vi "toString.vi"(10 "Variant":variant, 11 "StringFormatter in":refnum<class "StringFormatter.lvclass">) -> (2 "Value":string)   [LabVIEW 2013, in "OpenStringFormatter.lvlib" / "StringFormatter.lvclass"]
uses:
  StringFormatter.lvclass
  StringFormatter.lvclass/StringFormatter.ctl
  <vilib>/Utility/GetType.llb/TD_MDTFlavor.ctl
  TypeDescriptor/OpenDescriptor.lvlib
  Conversions/OpenConvert.lvlib
  Variant/OpenVariant.lvlib
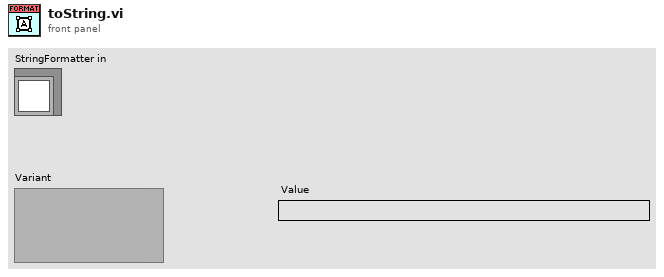
[diagram p1: front panel]
types:
  T1 = typedef "OpenStringFormatter.lvlib/StringFormatter.lvclass/Localization Decimal Separator -- enum.ctl" = enum16{"System", "Comma", "Dot"}
  T2 = typedef "VariantType.lvlib/UnitInfo.ctl" = cluster{"UnitType":T3, "Exponent":i16}
  T3 = typedef "VariantType.lvlib/UnitType.ctl" = enum16{"Radians", "Steradians", "Seconds", "Meters", "Kilograms", "Amperes", "Kelvins", "Moles", "Candelas", "InvalidUnit"}
  T4 = typedef "TD_Refnum Kind.ctl" = enum16{"Generic", "DataLog", "ByteStream", "Device", "Occur", "TCPNetConn", "OldVisa", "Auto", "LVObj", "Menu", "OldIVI", "Imaq", "Hardware", "DataSocket", "Visa", "IVI", "UDPNetConn", "Notifier", "Queue", "IrdaNetConn", "GenClass", "GenClassTag", "DAQMX", "EventReg", "DotNet", "UserEvent", "GenClassDeepCopy", "Callback", "GenClassFlatten", "GenClassTagFlatten", "LV Class Instance", "BtNetConn"}
  T5 = typedef "TD_MDTFlavor.ctl" = enum16{"kUnknown", "OldDblWaveform", "I16Waveform", "DBLWaveform", "Unused(4)", "SGLWaveform", "Timestamp", "DigitalTable", "DigitalWaveform", "Dynamic Express", "ExtWaveform", "U8Waveform", "U16Waveform", "U32Waveform", "I8Waveform", "I32Waveform", "CSGWaveform", "CDBWaveform", "CXTWaveform", "I64Waveform", "U64Waveform"}
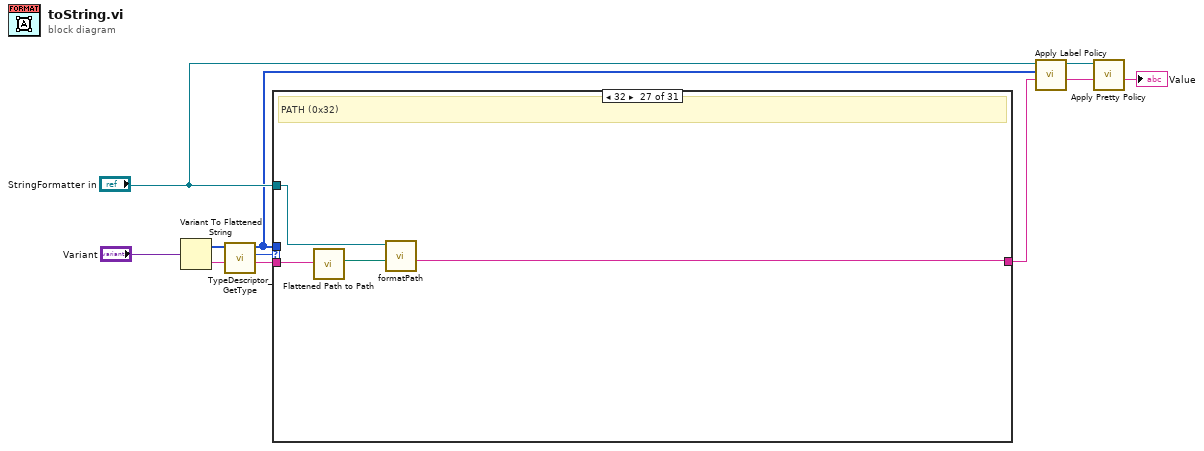
[diagram p0: block diagram]
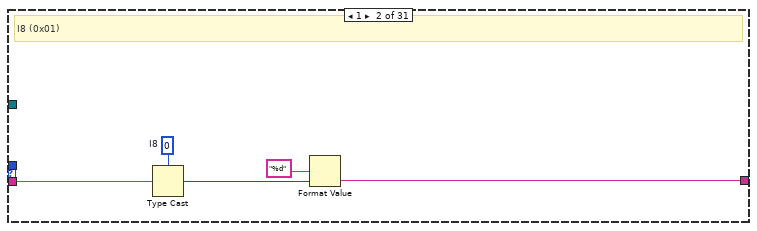
[diagram p3: hidden frame]
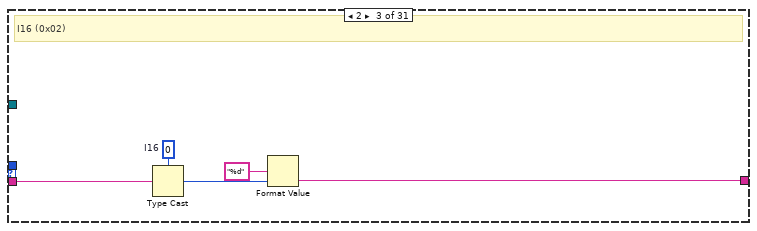
[diagram p4: hidden frame]
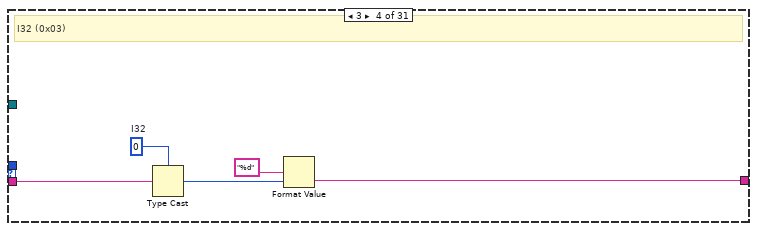
[diagram p5: hidden frame]
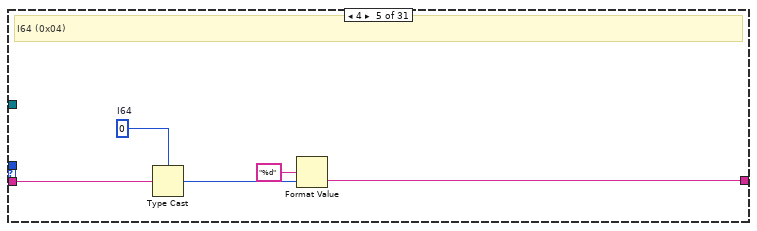
[diagram p6: hidden frame]
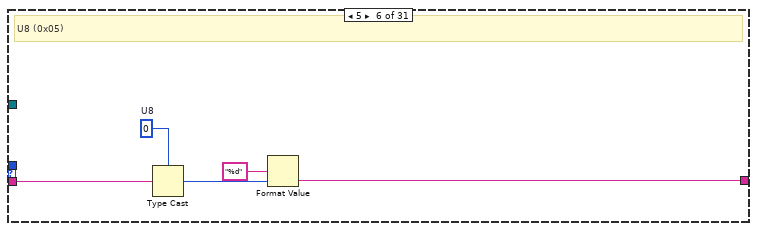
[diagram p7: hidden frame]
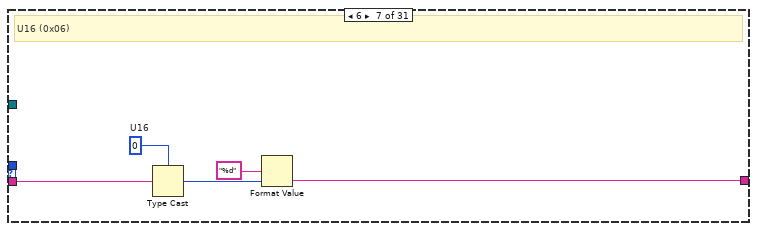
[diagram p8: hidden frame]
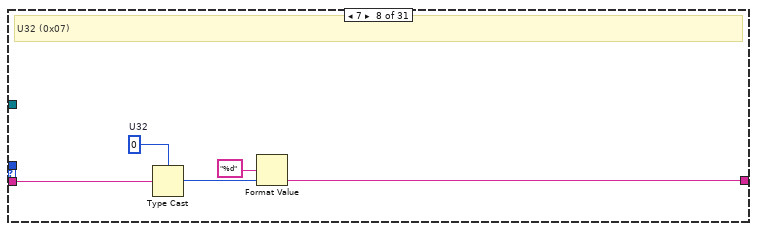
[diagram p9: hidden frame]
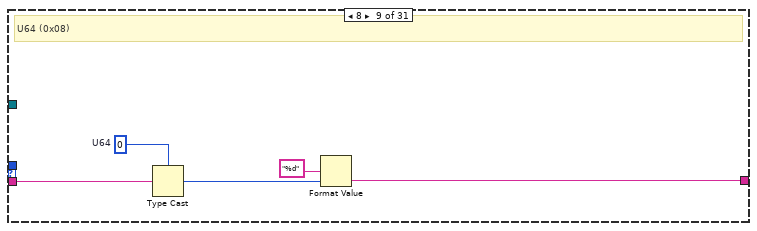
[diagram p10: hidden frame]
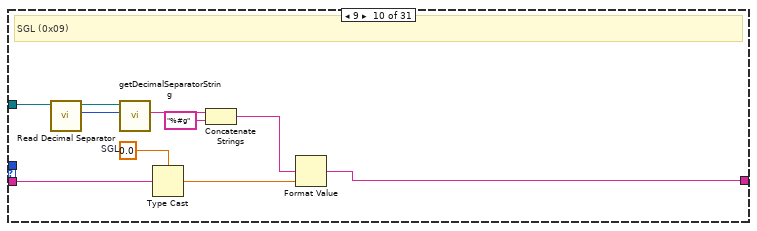
[diagram p11: hidden frame]
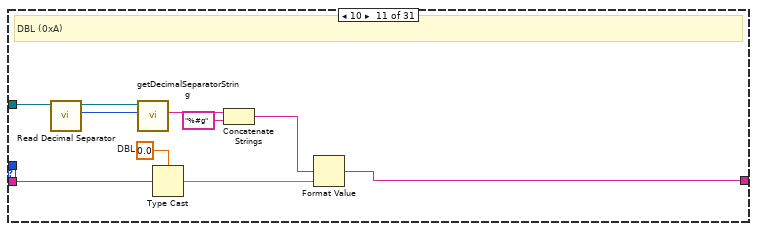
[diagram p12: hidden frame]
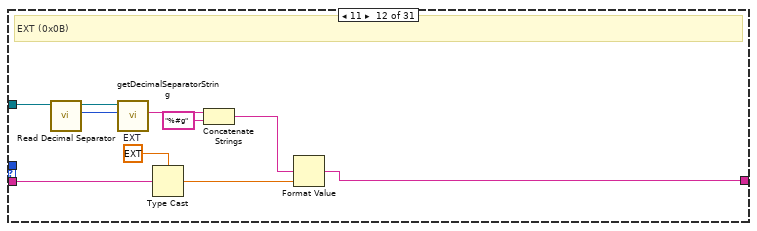
[diagram p13: hidden frame]
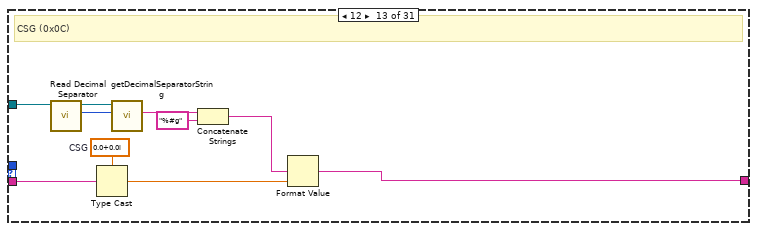
[diagram p14: hidden frame]
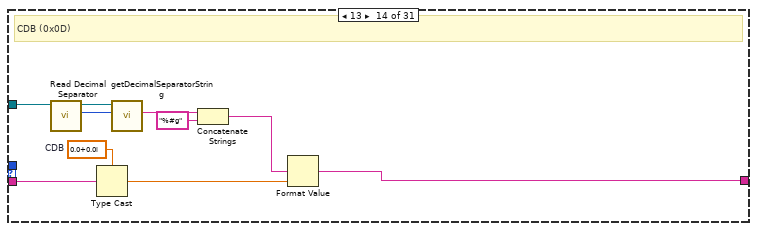
[diagram p15: hidden frame]
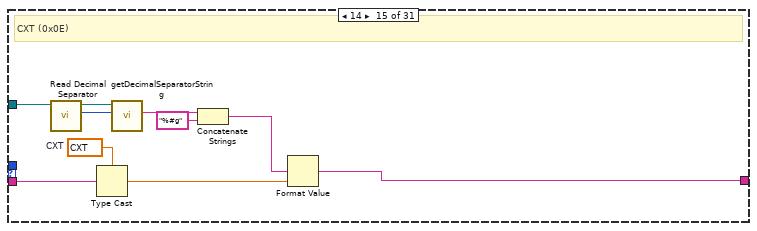
[diagram p16: hidden frame]
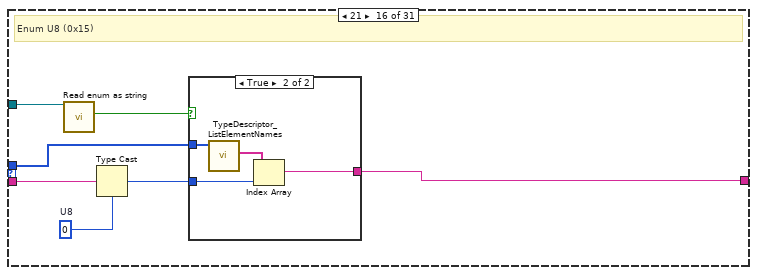
[diagram p17: hidden frame]
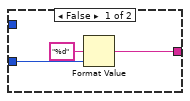
[diagram p18: hidden frame]
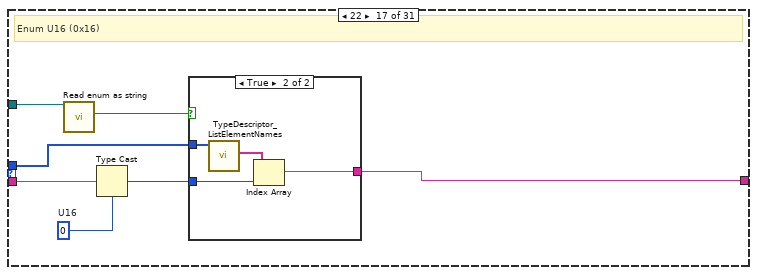
[diagram p19: hidden frame]
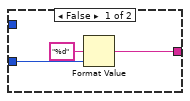
[diagram p20: hidden frame]
diagram:
  n1 = Variant To Flattened String(Variant="Variant") -> (data string=w8:string, 1:w10:i16[])
  n2 = call "TypeDescriptor_GetType.vi"("type descriptor"=w10) -> ("Type"=w9:u8, "type descriptor dup"=w5:i16[])  [unwired: 9 in]
  n3 = case shown="32" w9 {
    tunnel: [_ w11 w16 w21 w26 w31 w36 w41 w46 w52 w62 w72 w86 w97 w107 w115 w129 w143 w157 w173 w188 w203 w218 w233 w243 w250 w253 w257 w279 w303 w324] -> w4
    tunnel: w8 -> [_ w15 w19 w24 w29 w34 w39 w44 w49 w58 w69 w79 w89 w99 w109 w117 w131 w145 w167 w182 w197 w212 w227 w242 w248 w252 w256 w273 w291 w304 w325]
    tunnel: "StringFormatter in" -> [_ _ _ _ _ _ _ _ _ w59 w70 w80 w90 w100 w110 w113 w127 w140 w162 w178 w193 w208 w223 w238 _ w249 w254 w259 w281 w302 w323]
    tunnel: w5 -> [_ _ _ _ _ _ _ _ _ _ _ _ _ _ _ w114 w128 w141 w160 w176 w191 w206 w221 w236 _ _ _ w258 w280 w306 w322]
    frame 0, Default {
      # "Default"
    }
    frame 1 {
      w14 = i8 0  # I8
      # "I8 (0x01)"
      n4 = Type Cast(type=w14, x=w15) -> (*(type *) &x=w12:i8)
      n5 = Format Value(format string="%d", value (0)=w12) -> (output string=w11:string)  [unwired: 1 in]
    }
    frame 2 {
      w20 = i16 0  # I16
      # "I16 (0x02)"
      n6 = Type Cast(type=w20, x=w19) -> (*(type *) &x=w17:i16)
      n7 = Format Value(format string="%d", value (0)=w17) -> (output string=w16:string)  [unwired: 1 in]
    }
    frame 3 {
      w25 = 0  # I32
      # "I32 (0x03)"
      n8 = Type Cast(type=w25, x=w24) -> (*(type *) &x=w22:i32)
      n9 = Format Value(format string="%d", value (0)=w22) -> (output string=w21:string)  [unwired: 1 in]
    }
    frame 4 {
      w30 = i64 0  # I64
      # "I64 (0x04)"
      n10 = Type Cast(type=w30, x=w29) -> (*(type *) &x=w27:i64)
      n11 = Format Value(format string="%d", value (0)=w27) -> (output string=w26:string)  [unwired: 1 in]
    }
    frame 5 {
      w35 = u8 0  # U8
      # "U8 (0x05)"
      n12 = Type Cast(type=w35, x=w34) -> (*(type *) &x=w32:u8)
      n13 = Format Value(format string="%d", value (0)=w32) -> (output string=w31:string)  [unwired: 1 in]
    }
    frame 6 {
      w40 = u16 0  # U16
      # "U16 (0x06)"
      n14 = Type Cast(type=w40, x=w39) -> (*(type *) &x=w37:u16)
      n15 = Format Value(format string="%d", value (0)=w37) -> (output string=w36:string)  [unwired: 1 in]
    }
    frame 7 {
      w45 = u32 0  # U32
      # "U32 (0x07)"
      n16 = Type Cast(type=w45, x=w44) -> (*(type *) &x=w42:u32)
      n17 = Format Value(format string="%d", value (0)=w42) -> (output string=w41:string)  [unwired: 1 in]
    }
    frame 8 {
      w50 = u64 0  # U64
      # "U64 (0x08)"
      n18 = Type Cast(type=w50, x=w49) -> (*(type *) &x=w47:u64)
      n19 = Format Value(format string="%d", value (0)=w47) -> (output string=w46:string)  [unwired: 1 in]
    }
    frame 9 {
      w60 = sgl 0.0  # SGL
      # "SGL (0x09)"
      n20 = call "Read Decimal Separator.vi"("StringFormatter in"=w59) -> ("Decimal Separator"=w54:T1, "StringFormatter out"=w51:refnum<class "StringFormatter.lvclass">)  [unwired: 9 in]
      n21 = call-dynamic "getDecimalSeparatorString.vi"("Decimal Separator"=w54, "StringFormatter"=w51) -> ("Formatter String"=w57:string)  [unwired: 9 in]
      n22 = Type Cast(type=w60, x=w58) -> (*(type *) &x=w53:sgl)
      n23 = Concatenate Strings(w57, "%#g" ("string")) -> (w56:string)
      n24 = Format Value(format string=w56, value (0)=w53) -> (output string=w52:string)  [unwired: 1 in]
    }
    frame 10 {
      w68 = 0.0  # DBL
      # "DBL (0xA)"
      n25 = call "Read Decimal Separator.vi"("StringFormatter in"=w70) -> ("Decimal Separator"=w64:T1, "StringFormatter out"=w61:refnum<class "StringFormatter.lvclass">)  [unwired: 9 in]
      n26 = call-dynamic "getDecimalSeparatorString.vi"("Decimal Separator"=w64, "StringFormatter"=w61) -> ("Formatter String"=w67:string)  [unwired: 9 in]
      n27 = Type Cast(type=w68, x=w69) -> (*(type *) &x=w63:dbl)
      n28 = Concatenate Strings(w67, "%#g" ("string")) -> (w66:string)
      n29 = Format Value(format string=w66, value (0)=w63) -> (output string=w62:string)  [unwired: 1 in]
    }
    frame 11 {
      w78 = ext 0.0  # EXT
      # "EXT (0x0B)"
      n30 = call "Read Decimal Separator.vi"("StringFormatter in"=w80) -> ("Decimal Separator"=w74:T1, "StringFormatter out"=w71:refnum<class "StringFormatter.lvclass">)  [unwired: 9 in]
      n31 = call-dynamic "getDecimalSeparatorString.vi"("Decimal Separator"=w74, "StringFormatter"=w71) -> ("Formatter String"=w77:string)  [unwired: 9 in]
      n32 = Type Cast(type=w78, x=w79) -> (*(type *) &x=w73:ext)
      n33 = Concatenate Strings(w77, "%#g" ("string")) -> (w76:string)
      n34 = Format Value(format string=w76, value (0)=w73) -> (output string=w72:string)  [unwired: 1 in]
    }
    frame 12 {
      w88 = csg 0.0+0.0i  # CSG
      # "CSG (0x0C)"
      n35 = call "Read Decimal Separator.vi"("StringFormatter in"=w90) -> ("Decimal Separator"=w85:T1, "StringFormatter out"=w81:refnum<class "StringFormatter.lvclass">)  [unwired: 9 in]
      n36 = Type Cast(type=w88, x=w89) -> (*(type *) &x=w87:csg)
      n37 = call-dynamic "getDecimalSeparatorString.vi"("Decimal Separator"=w85, "StringFormatter"=w81) -> ("Formatter String"=w84:string)  [unwired: 9 in]
      n38 = Concatenate Strings(w84, "%#g" ("string")) -> (w83:string)
      n39 = Format Value(format string=w83, value (0)=w87) -> (output string=w86:string)  [unwired: 1 in]
    }
    frame 13 {
      w92 = cdb 0.0+0.0i  # CDB
      # "CDB (0x0D)"
      n40 = call "Read Decimal Separator.vi"("StringFormatter in"=w100) -> ("Decimal Separator"=w96:T1, "StringFormatter out"=w91:refnum<class "StringFormatter.lvclass">)  [unwired: 9 in]
      n41 = Type Cast(type=w92, x=w99) -> (*(type *) &x=w98:cdb)
      n42 = call-dynamic "getDecimalSeparatorString.vi"("Decimal Separator"=w96, "StringFormatter"=w91) -> ("Formatter String"=w95:string)  [unwired: 9 in]
      n43 = Concatenate Strings(w95, "%#g" ("string")) -> (w94:string)
      n44 = Format Value(format string=w94, value (0)=w98) -> (output string=w97:string)  [unwired: 1 in]
    }
    frame 14 {
      w102 = cxt 0.0+0.0i  # CXT
      # "CXT (0x0E)"
      n45 = call "Read Decimal Separator.vi"("StringFormatter in"=w110) -> ("Decimal Separator"=w106:T1, "StringFormatter out"=w101:refnum<class "StringFormatter.lvclass">)  [unwired: 9 in]
      n46 = Type Cast(type=w102, x=w109) -> (*(type *) &x=w108:cxt)
      n47 = call-dynamic "getDecimalSeparatorString.vi"("Decimal Separator"=w106, "StringFormatter"=w101) -> ("Formatter String"=w105:string)  [unwired: 9 in]
      n48 = Concatenate Strings(w105, "%#g" ("string")) -> (w104:string)
      n49 = Format Value(format string=w104, value (0)=w108) -> (output string=w107:string)  [unwired: 1 in]
    }
    frame 21 {
      w111 = u8 0  # U8
      # "Enum U8 (0x15)"
      n50 = call "Read enum as string.vi"("StringFormatter in"=w113) -> ("enum as string"=w112:bool)  [unwired: 9 in, 1 out]
      n51 = Type Cast(type=w111, x=w117) -> (*(type *) &x=w116:u8)
      n52 = case shown="True" w112 {
        tunnel: w116 -> [w120 w122]
        tunnel: [w119 w121] -> w115
        tunnel: w114 -> [_ w124]
        frame False {
          n53 = Format Value(format string="%d", value (0)=w120) -> (output string=w119:string)  [unwired: 1 in]
        }
        frame True {
          n54 = call "TypeDescriptor_ListElementNames.vi"("type descriptor"=w124) -> ("element names"=w123:string[])  [unwired: 7 in, 3 out]
          n55 = Index Array(array=w123, index=w122) -> (element=w121:string)
        }
      }
    }
    frame 22 {
      w125 = u16 0  # U16
      # "Enum U16 (0x16)"
      n56 = call "Read enum as string.vi"("StringFormatter in"=w127) -> ("enum as string"=w126:bool)  [unwired: 9 in, 1 out]
      n57 = Type Cast(type=w125, x=w131) -> (*(type *) &x=w130:u16)
      n58 = case shown="True" w126 {
        tunnel: w130 -> [w134 w136]
        tunnel: [w133 w135] -> w129
        tunnel: w128 -> [_ w138]
        frame False {
          n59 = Format Value(format string="%d", value (0)=w134) -> (output string=w133:string)  [unwired: 1 in]
        }
        frame True {
          n60 = call "TypeDescriptor_ListElementNames.vi"("type descriptor"=w138) -> ("element names"=w137:string[])  [unwired: 7 in, 3 out]
          n61 = Index Array(array=w137, index=w136) -> (element=w135:string)
        }
      }
    }
    frame 23 {
      w142 = u32 0  # U32
      # "Enum U32 (0x17)"
      n62 = call "Read enum as string.vi"("StringFormatter in"=w140) -> ("enum as string"=w139:bool)  [unwired: 9 in, 1 out]
      n63 = Type Cast(type=w142, x=w145) -> (*(type *) &x=w144:u32)
      n64 = case shown="True" w139 {
        tunnel: w144 -> [w148 w150]
        tunnel: [w147 w149] -> w143
        tunnel: w141 -> [_ w152]
        frame False {
          n65 = Format Value(format string="%d", value (0)=w148) -> (output string=w147:string)  [unwired: 1 in]
        }
        frame True {
          n66 = call "TypeDescriptor_ListElementNames.vi"("type descriptor"=w152) -> ("element names"=w151:string[])  [unwired: 7 in, 3 out]
          n67 = Index Array(array=w151, index=w150) -> (element=w149:string)
        }
      }
    }
    frame 25 {
      w165 = sgl 0.0  # SGL
      # "SGL PhysUnit (0x19)"
      n68 = call "Read Decimal Separator.vi"("StringFormatter in"=w162) -> ("Decimal Separator"=w161:T1, "StringFormatter out"=w153:refnum<class "StringFormatter.lvclass">)  [unwired: 9 in]
      n69 = call "TypeDescriptor_GetUnits.vi"("type descriptor"=w160) -> ("Units"=w155:T2[])  [unwired: 8 in, 2 out]
      n70 = Type Cast(type=w165, x=w167) -> (*(type *) &x=w166:sgl)
      n71 = call-dynamic "formatUnits.vi"("Units"=w155, "StringFormatter"=w153) -> ("Units String"=w154:string)  [unwired: 9 in]
      n72 = call-dynamic "getDecimalSeparatorString.vi"("Decimal Separator"=w161, "StringFormatter"=w153) -> ("Formatter String"=w164:string)  [unwired: 9 in]
      n73 = Concatenate Strings(w164, "%#g" ("string")) -> (w159:string)
      n74 = Format Value(format string=w159, value (0)=w166) -> (output string=w158:string)  [unwired: 1 in]
      n75 = call <vilib>:"Space Constant.vi"() -> ("String"=w156:string)
      n76 = Concatenate Strings(w158, w156, w154) -> (w157:string)
    }
    frame 26 {
      w168 = 0.0  # DBL
      # "DBL PhysUnit (0x1A)"
      n77 = call "Read Decimal Separator.vi"("StringFormatter in"=w178) -> ("Decimal Separator"=w177:T1, "StringFormatter out"=w169:refnum<class "StringFormatter.lvclass">)  [unwired: 9 in]
      n78 = call "TypeDescriptor_GetUnits.vi"("type descriptor"=w176) -> ("Units"=w171:T2[])  [unwired: 8 in, 2 out]
      n79 = Type Cast(type=w168, x=w182) -> (*(type *) &x=w181:dbl)
      n80 = call-dynamic "formatUnits.vi"("Units"=w171, "StringFormatter"=w169) -> ("Units String"=w170:string)  [unwired: 9 in]
      n81 = call-dynamic "getDecimalSeparatorString.vi"("Decimal Separator"=w177, "StringFormatter"=w169) -> ("Formatter String"=w180:string)  [unwired: 9 in]
      n82 = Concatenate Strings(w180, "%#g" ("string")) -> (w175:string)
      n83 = Format Value(format string=w175, value (0)=w181) -> (output string=w174:string)  [unwired: 1 in]
      n84 = call <vilib>:"Space Constant.vi"() -> ("String"=w172:string)
      n85 = Concatenate Strings(w174, w172, w170) -> (w173:string)
    }
    frame 27 {
      w183 = ext 0.0  # EXT
      # "EXT PhysUnit (0x1B)"
      n86 = call "Read Decimal Separator.vi"("StringFormatter in"=w193) -> ("Decimal Separator"=w192:T1, "StringFormatter out"=w184:refnum<class "StringFormatter.lvclass">)  [unwired: 9 in]
      n87 = call "TypeDescriptor_GetUnits.vi"("type descriptor"=w191) -> ("Units"=w186:T2[])  [unwired: 8 in, 2 out]
      n88 = Type Cast(type=w183, x=w197) -> (*(type *) &x=w196:ext)
      n89 = call-dynamic "formatUnits.vi"("Units"=w186, "StringFormatter"=w184) -> ("Units String"=w185:string)  [unwired: 9 in]
      n90 = call-dynamic "getDecimalSeparatorString.vi"("Decimal Separator"=w192, "StringFormatter"=w184) -> ("Formatter String"=w195:string)  [unwired: 9 in]
      n91 = Concatenate Strings(w195, "%#g" ("string")) -> (w190:string)
      n92 = Format Value(format string=w190, value (0)=w196) -> (output string=w189:string)  [unwired: 1 in]
      n93 = call <vilib>:"Space Constant.vi"() -> ("String"=w187:string)
      n94 = Concatenate Strings(w189, w187, w185) -> (w188:string)
    }
    frame 28 {
      w198 = csg 0.0+0.0i  # CSG
      # "CSG PhysUnit (0x1C)"
      n95 = call "Read Decimal Separator.vi"("StringFormatter in"=w208) -> ("Decimal Separator"=w207:T1, "StringFormatter out"=w199:refnum<class "StringFormatter.lvclass">)  [unwired: 9 in]
      n96 = call "TypeDescriptor_GetUnits.vi"("type descriptor"=w206) -> ("Units"=w201:T2[])  [unwired: 8 in, 2 out]
      n97 = Type Cast(type=w198, x=w212) -> (*(type *) &x=w211:csg)
      n98 = call-dynamic "formatUnits.vi"("Units"=w201, "StringFormatter"=w199) -> ("Units String"=w200:string)  [unwired: 9 in]
      n99 = call-dynamic "getDecimalSeparatorString.vi"("Decimal Separator"=w207, "StringFormatter"=w199) -> ("Formatter String"=w210:string)  [unwired: 9 in]
      n100 = Concatenate Strings(w210, "%#g" ("string")) -> (w205:string)
      n101 = Format Value(format string=w205, value (0)=w211) -> (output string=w204:string)  [unwired: 1 in]
      n102 = call <vilib>:"Space Constant.vi"() -> ("String"=w202:string)
      n103 = Concatenate Strings(w204, w202, w200) -> (w203:string)
    }
    frame 29 {
      w213 = cdb 0.0+0.0i  # CDB
      # "CDB PhysUnit (0x1D)"
      n104 = call "Read Decimal Separator.vi"("StringFormatter in"=w223) -> ("Decimal Separator"=w222:T1, "StringFormatter out"=w214:refnum<class "StringFormatter.lvclass">)  [unwired: 9 in]
      n105 = call "TypeDescriptor_GetUnits.vi"("type descriptor"=w221) -> ("Units"=w216:T2[])  [unwired: 8 in, 2 out]
      n106 = Type Cast(type=w213, x=w227) -> (*(type *) &x=w226:cdb)
      n107 = call-dynamic "formatUnits.vi"("Units"=w216, "StringFormatter"=w214) -> ("Units String"=w215:string)  [unwired: 9 in]
      n108 = call-dynamic "getDecimalSeparatorString.vi"("Decimal Separator"=w222, "StringFormatter"=w214) -> ("Formatter String"=w225:string)  [unwired: 9 in]
      n109 = Concatenate Strings(w225, "%#g" ("string")) -> (w220:string)
      n110 = Format Value(format string=w220, value (0)=w226) -> (output string=w219:string)  [unwired: 1 in]
      n111 = call <vilib>:"Space Constant.vi"() -> ("String"=w217:string)
      n112 = Concatenate Strings(w219, w217, w215) -> (w218:string)
    }
    frame 30 {
      w228 = cxt 0.0+0.0i  # CXT
      # "CXT PhysUnit (0x1E)"
      n113 = call "Read Decimal Separator.vi"("StringFormatter in"=w238) -> ("Decimal Separator"=w237:T1, "StringFormatter out"=w229:refnum<class "StringFormatter.lvclass">)  [unwired: 9 in]
      n114 = call "TypeDescriptor_GetUnits.vi"("type descriptor"=w236) -> ("Units"=w231:T2[])  [unwired: 8 in, 2 out]
      n115 = Type Cast(type=w228, x=w242) -> (*(type *) &x=w241:cxt)
      n116 = call-dynamic "formatUnits.vi"("Units"=w231, "StringFormatter"=w229) -> ("Units String"=w230:string)  [unwired: 9 in]
      n117 = call-dynamic "getDecimalSeparatorString.vi"("Decimal Separator"=w237, "StringFormatter"=w229) -> ("Formatter String"=w240:string)  [unwired: 9 in]
      n118 = Concatenate Strings(w240, "%#g" ("string")) -> (w235:string)
      n119 = Format Value(format string=w235, value (0)=w241) -> (output string=w234:string)  [unwired: 1 in]
      n120 = call <vilib>:"Space Constant.vi"() -> ("String"=w232:string)
      n121 = Concatenate Strings(w234, w232, w230) -> (w233:string)
    }
    frame 33 {
      # "Boolean (0x21)"
      n122 = Type Cast(type=FALSE, x=w248) -> (*(type *) &x=w246:bool)
      n123 = Select(t="true", s=w246, f="false") -> (s? t:f=w243:string)
    }
    frame 48 {
      # "STRING (0x30)"
      n124 = call "Flattened String to String.vi"("Flattened String"=w252) -> ("String"=w251:string)  [unwired: 9 in, 1 out]
      n125 = call-dynamic "formatString.vi"("Value"=w251, "StringFormatter"=w249) -> ("Formatted Value"=w250:string)  [unwired: 9 in]
    }
    frame 50 {
      # "PATH (0x32)"
      n126 = call "Flattened Path to Path.vi"("Flattened Path String"=w256) -> ("path"=w255:path)  [unwired: 10 in]
      n127 = call-dynamic "formatPath.vi"("Value"=w255, "StringFormatter"=w254) -> ("Formatted Value"=w253:string)  [unwired: 9 in]
    }
    frame 64 {
      # "ARRAY (0x40)"
      n128 = call "Write quoted string.vi"("quoted string"=TRUE, "StringFormatter in"=w259) -> ("StringFormatter out"=w261:refnum<class "StringFormatter.lvclass">)  [unwired: 9 in]
      n129 = call "Flattened Array to Flattened Elements.vi"("Flattened Array String"=w273, "Array Type Descriptor"=w258) -> ("Flattened Array Elements"=w271:string[], "Array Element Type Descriptor"=w272:i16[])  [unwired: 8 in]
      n130 = call "Write label.vi"("label"=FALSE, "StringFormatter in"=w261) -> ("StringFormatter out"=w260:refnum<class "StringFormatter.lvclass">)  [unwired: 9 in]
      n131 = for {
        tunnel: w260 -> [w275]
        tunnel: w272 -> [w278]
        tunnel: w271 -> [w277] mode=indexing
        tunnel: [w274] -> w270 mode=indexing
        n132 = Flattened String To Variant(6:w277, 7:w278) -> (3:w276:variant)  [unwired: 1 in, 1 out]
        n133 = call "Variant_FormatToString.vi"("Formatter"=w275, "Variant"=w276) -> ("Value"=w274:string)  [unwired: 9 in]
      }
      n134 = Array To Spreadsheet String(delimiter (Tab)=",", array=w270, 3:"" ("format string")) -> (spreadsheet string=w267:string)
      n135 = call <vilib>:"Trim Whitespace.vi"("string"=w267) -> ("trimmed string"=w266:string)  [unwired: 1 in]
      n136 = Concatenate Strings("[", w266, "]") -> (w257:string)
    }
    frame 80 {
      # "CLUSTER (0x50)"
      n137 = call "Write quoted string.vi"("quoted string"=TRUE, "StringFormatter in"=w281) -> ("StringFormatter out"=w287:refnum<class "StringFormatter.lvclass">)  [unwired: 9 in]
      n138 = call "Flattened Cluster to Flattened Elements.vi"("Flattened Cluster"=w291, "Cluster Type Descriptor"=w280) -> ("Flattened Cluster Elements"=w289:string[], "Elements Type Descriptor"=w290:cluster{"Type Descriptor":i16[]}[])  [unwired: 8 in]
      n139 = call "Write label.vi"("label"=TRUE, "StringFormatter in"=w287) -> ("StringFormatter out"=w282:refnum<class "StringFormatter.lvclass">)  [unwired: 9 in]
      n140 = for {
        tunnel: w282 -> [w297]
        tunnel: w290 -> [w300] mode=indexing
        tunnel: w289 -> [w301] mode=indexing
        tunnel: [w296] -> w295 mode=indexing
        n141 = Unbundle(w300) -> ("Type Descriptor"=w299:i16[])
        n142 = Flattened String To Variant(6:w301, 7:w299) -> (3:w298:variant)  [unwired: 1 in, 1 out]
        n143 = call "Variant_FormatToString.vi"("Formatter"=w297, "Variant"=w298) -> ("Value"=w296:string)  [unwired: 9 in]
      }
      n144 = Array To Spreadsheet String(delimiter (Tab)=",", array=w295, 3:"" ("format string")) -> (spreadsheet string=w292:string)
      n145 = call <vilib>:"Trim Whitespace.vi"("string"=w292) -> ("trimmed string"=w283:string)  [unwired: 1 in]
      n146 = Concatenate Strings("{", w283, "}") -> (w279:string)
    }
    frame 112 {
      # "REFNUMS (0x70)"
      n147 = call <vilib>:"TD_Get Ref Info.vi"("Type descriptor"=w306) -> ("Refnum Type"=w305:T4)  [unwired: 10 in]
      n148 = case shown="\"Generic\", Default" w305 {
        tunnel: w306 -> [_ _ w319]
        tunnel: w304 -> [w310 w315 _]
        tunnel: [w307 w312 w316] -> w303
        tunnel: w302 -> [_ w314 w318]
        frame "Generic", Default {
          # "Generic Refnum"
          n149 = Type Cast(type=u32 0, x=w310) -> (*(type *) &x=w308:u32)
          n150 = Format Value(format string="0x%04x", value (0)=w308) -> (output string=w307:string)  [unwired: 1 in]
        }
        frame "Visa", "IVI", "GenClassTag", "DAQMX" {
          # "VISA, GenericClassTag, IVI, DAQmx"
          n151 = call "Flattened String to String.vi"("Flattened String"=w315) -> ("String"=w313:string)  [unwired: 9 in, 1 out]
          n152 = call-dynamic "formatString.vi"("Value"=w313, "StringFormatter"=w314) -> ("Formatted Value"=w312:string)  [unwired: 9 in]
        }
        frame "LV Class Instance" {
          # "Class Instance"
          n153 = call <vilib>:"TD_Get LVClass Info.vi"("Type descriptor"=w319) -> ("LV Class File Name"=w317:string)  [unwired: 9 in, 1 out]
          n154 = call-dynamic "formatString.vi"("Value"=w317, "StringFormatter"=w318) -> ("Formatted Value"=w316:string)  [unwired: 9 in]
        }
      }
    }
    frame 84 {
      (unwired) TD_MDTFlavor."Timestamp" ("MDT Flavor")
      # "WAVEFORMS (0x54)"
      n155 = call <vilib>:"TD_Get MDT Information.vi"("Type descriptor"=w322) -> ("Contained Cluster Offset"=w320:i32, "MDT Flavor"=w321:T5)  [unwired: 9 in]
      n156 = case shown="\"Timestamp\"" w321 {
        tunnel: w322 -> [_ w330]
        tunnel: w325 -> [_ w329]
        tunnel: [_ w327] -> w324
        tunnel: w323 -> [_ w328]
        tunnel: w320 -> [_ _]
        frame Default {
          # "Unknown"
        }
        frame "Timestamp" {
          # "Timestamp"
          n157 = Flattened String To Variant(6:w329, 7:w330) -> (3:w332:variant)  [unwired: 1 in, 1 out]
          n158 = Variant To Data(type=timestamp(0 s since 1904-01-01) ("current time"), Variant=w332) -> (data=w326:timestamp)  [unwired: 1 in, 1 out]
          n159 = call-dynamic "formatTimestamp.vi"("Value"=w326, "StringFormatter"=w328) -> ("Formatted Value"=w327:string)  [unwired: 9 in]
        }
      }
    }
  }
  n160 = call "Apply Label Policy.vi"("String"=w4, "type descriptor"=w5, "StringFormatter"="StringFormatter in") -> ("Labeled String"=w2:string, "StringFormatter out"=w3:refnum<class "StringFormatter.lvclass">)  [unwired: 7 in]
  n161 = call "Apply Pretty Policy.vi"("String"=w2, "StringFormatter"=w3) -> ("Pretty String"=→"Value":string)  [unwired: 8 in, 1 out]
